vi "Clamp Demo.vi"() -> ()   [LabVIEW 2026]
doc: "Two-VI program: a While loop accumulates Increment onto Start Value each iteration, passes the candidate through the Clamp Value.vi subVI to hold it inside [Lower Bound, Upper Bound], counts iterations, flags whether any value ever left the range, and collects the per-iteration clamped history as an array. The loop stops once the iteration count reaches Max Iterations."
panel:
  out "History":dbl[](array[numeric])
  out "Saturated":bool
  out "Iterations":i32
  out "Final Value":dbl
  in  "Max Iterations":i32=8
  in  "Upper Bound":dbl=10.0
  in  "Lower Bound":dbl
  in  "Increment":dbl=1.5
  in  "Start Value":dbl
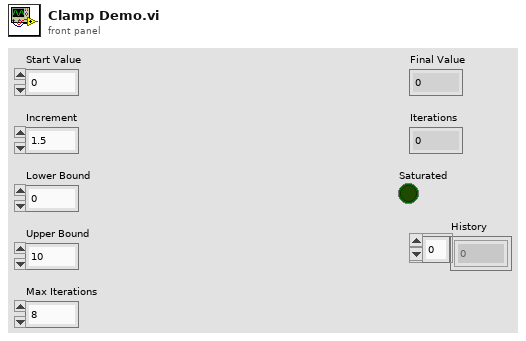
[diagram p1: front panel]
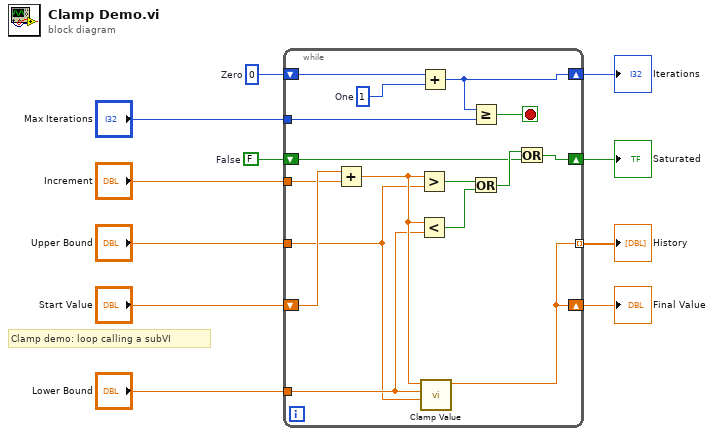
[diagram p0: block diagram]
diagram:
  w5 = FALSE  # False
  w6 = 0  # Zero
  # "Clamp demo: loop calling a subVI"
  n1 = while {
    tunnel: "Increment" -> [w26]
    tunnel: "Lower Bound" -> [w17]
    tunnel: "Upper Bound" -> [w16]
    tunnel: "Max Iterations" -> [w20]
    shift-right: [w12] -> w4
    shift-left: "Start Value" -> [w27]
    shift-right: [w21] -> w3
    shift-left: w6 -> [w23]
    shift-right: [w13] -> w2
    shift-left: w5 -> [w14]
    tunnel: [w12] -> w1 mode=indexing
    stop <- w19 stop-if-true
    w22 = 1  # One
    n2 = Add(x=w27, y=w26) -> (x+y=w18:dbl)
    n3 = Greater?(x=w18, y=w16) -> (0:w25:bool)
    n4 = Less?(x=w18, y=w17) -> (x < y?=w24:bool)
    n5 = Add(x=w23, y=w22) -> (x+y=w21:i32)
    n6 = call "Clamp Value.vi"("hi"=w16, "lo"=w17, "x"=w18) -> ("clamped"=w12:dbl)  [unwired: 8 in]
    n7 = Greater Or Equal?(x=w21, y=w20) -> (x >= y?=w19:bool)
    n8 = Or(x=w25, y=w24) -> (x .or. y?=w15:bool)
    n9 = Or(x=w15, y=w14) -> (x .or. y?=w13:bool)
  }
  "Final Value" <- w4
  "Iterations" <- w3
  "Saturated" <- w2
  "History" <- w1
